vi "PicoScope2000Stop.vi"(8 "error in (no error)":errorcluster, 11 "handle in":i16=16384) -> (0 "error out":errorcluster, 3 "handle out":i16)   [LabVIEW 2010]
doc: "This stops the device capturing data and should be called before retrieving data from the device."
uses:
  ps2000.dll
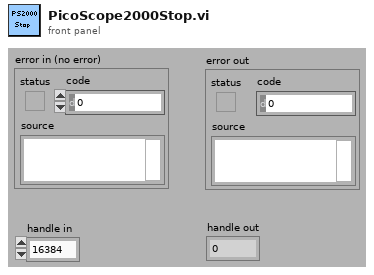
[diagram p1: front panel]
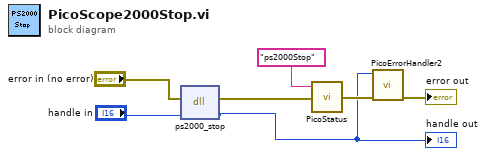
[diagram p0: block diagram]
diagram:
  n1 = dll-call lib="PS2000.dll" fn="ps2000_stop"(error in="error in (no error)", "handle"="handle in") -> (error out=w2:errorcluster, "handle"=w1:i16)  [unwired: 3 in, 1 out]
  "handle out" <- w1
  n2 = call "PicoStatus.vi"("error in"=w2, "source"="ps2000Stop") -> ("error out"=w7:errorcluster)  [unwired: 1 in]
  n3 = call "PicoErrorHandler2.vi"("error in (no error)"=w7, "handle In"=w1) -> ("error out"=→"error out":errorcluster)  [unwired: 9 in]
